vi "Modbus_RTU_Battery.vi"(0 "STOP":bool, 1 "High Volt alarm (0.01V)":string, 2 "error in":errorcluster, 3 "Low Volt alarm (0.01V)":string, 4 "Modbus RTU Address":string, 5 "Currrent Range":string(combo), 6 "VISA resource name":refnum<visa-resource-name>, 7 "baud rate":u32=9600) -> (11 "HighAlarm":bool, 13 "LowAlarm":bool, 14 "Voltage(V)":dbl, 15 "Current(A)":dbl, 16 "error out":errorcluster, 17 "Energy(Wh)":dbl, 18 "Power(W)":dbl, 19 "ChangeDone":bool)   [LabVIEW 2025]
uses:
  <vilib>/NI/Modbus Library/API/Wrapper/Create Serial Master.vi
  <vilib>/NI/Modbus Library/API/Master/Modbus Master.lvclass
  <vilib>/NI/Modbus Library/API/Wrapper/API Main.lvlib
panel:
  out "register parameter":u16[](array[numeric])
  out "register data":u16[](array[numeric])
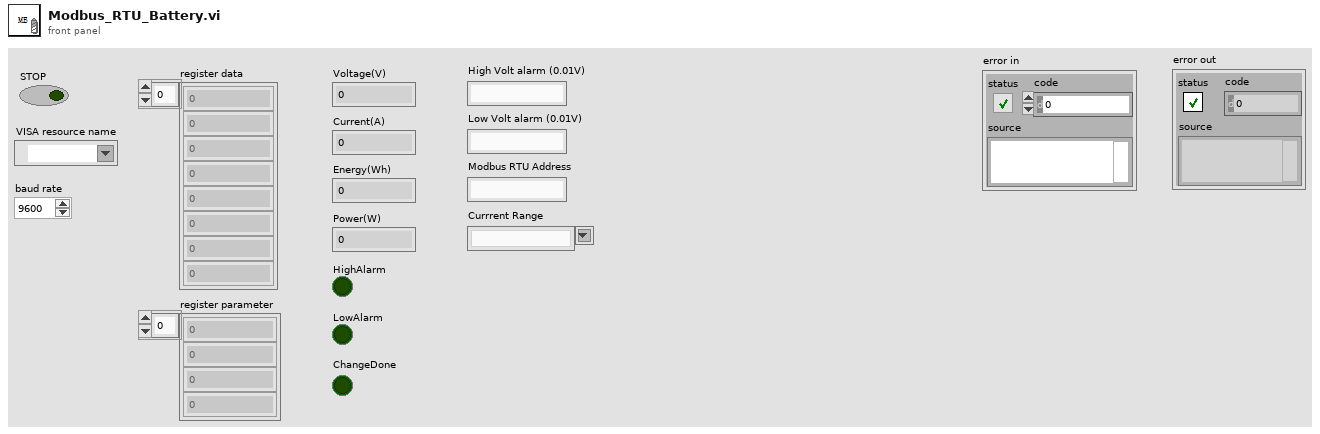
[diagram p1: front panel]
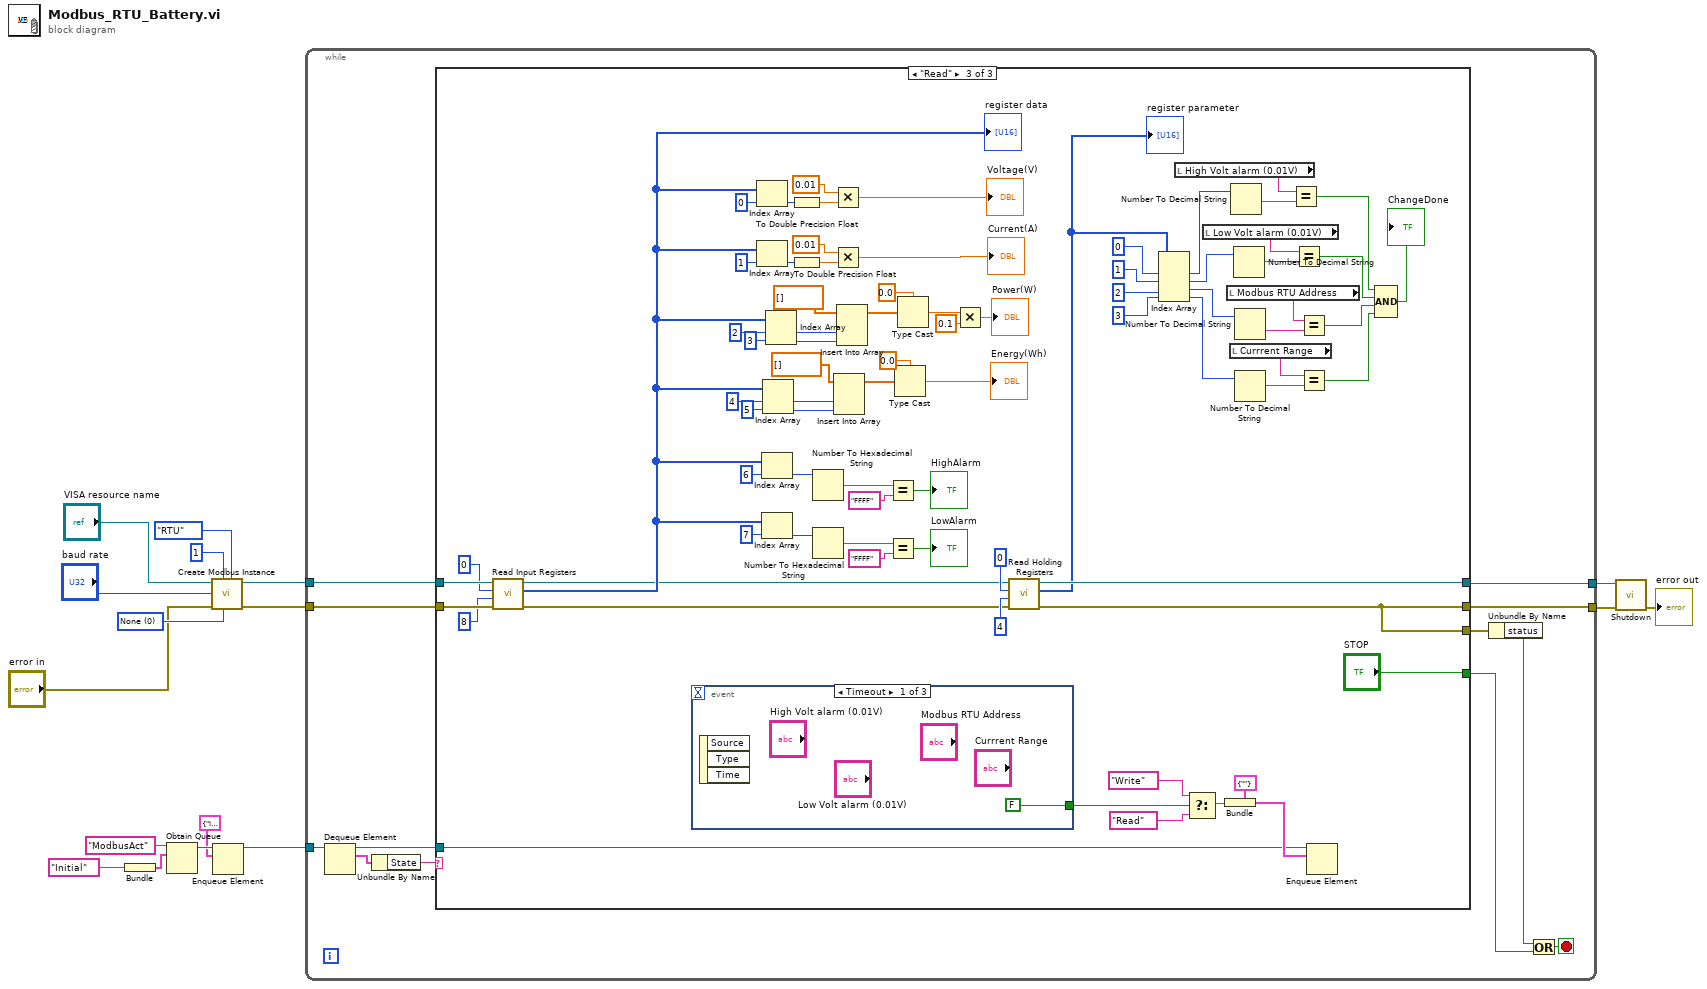
[diagram p0: block diagram]
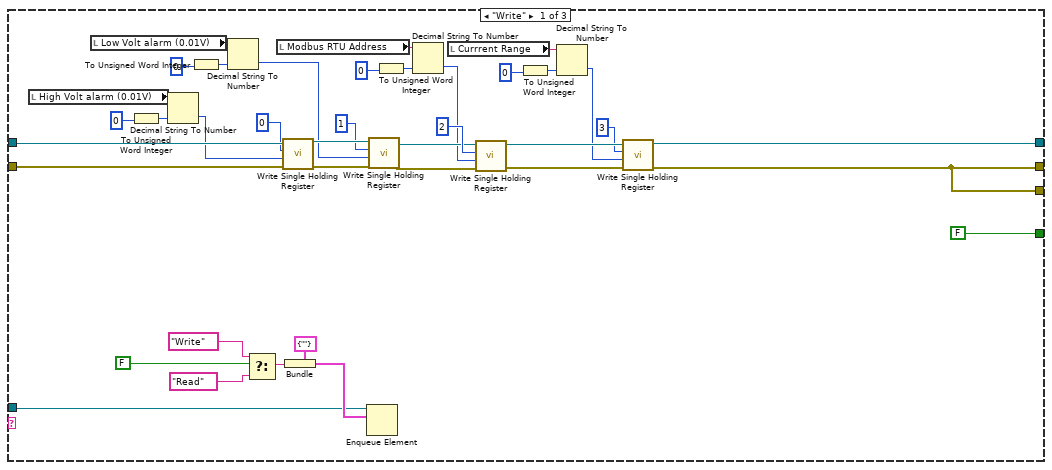
[diagram p2: hidden frame]
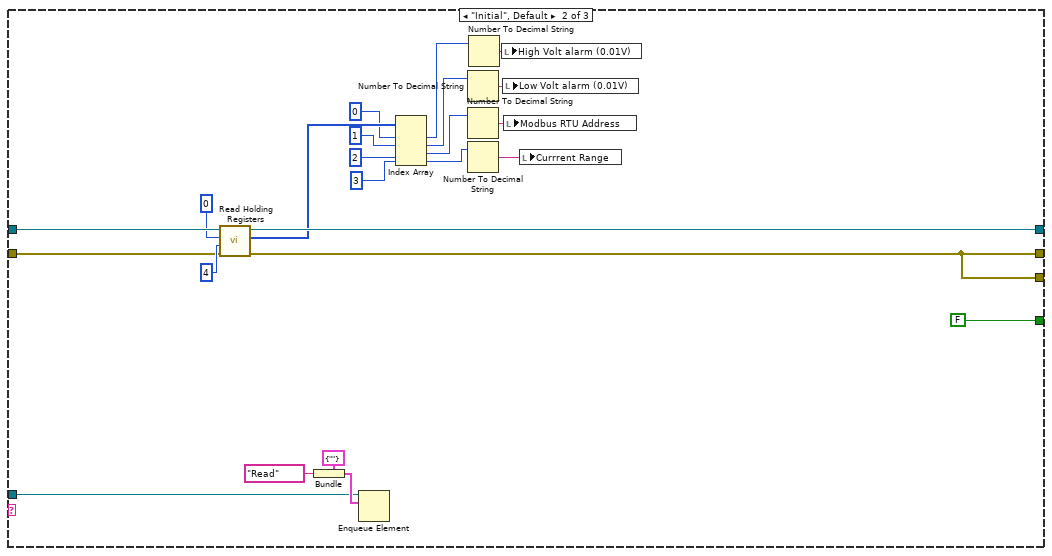
[diagram p3: hidden frame]
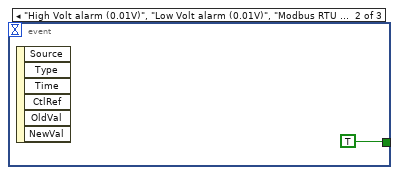
[diagram p4: hidden frame]
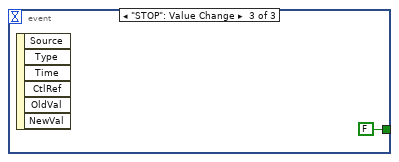
[diagram p5: hidden frame]
diagram:
  w15 = u16 0 items=["None", "Odd", "Even", "Mark", "Space"] ("parity (even)")
  n1 = Bundle("State"="Initial") -> (w6:cluster{"State":string})  [unwired: 1 in]
  n2 = Obtain Queue(name (unnamed)="ModbusAct" ("名称（未命名）"), element data type=w6) -> (queue out=w10:refnum<queue>)  [unwired: 3 in, 2 out]
  n3 = call-poly <vilib>:"Create Modbus Instance.vi"("serial type"=enum16{"RTU", "ASCII"}."RTU", "parity (even)"=w15, "unit ID"=u8 1, "error in"="error in", "baud rate"="baud rate", "VISA resource name"="VISA resource name") -> ("error out"=w13:errorcluster, "serial master instance"=w14:refnum<class "Modbus Master.lvclass">)  [unwired: 4 in]
  n4 = Enqueue Element(queue=w10, element=cluster{string} {"Initial"}) -> (queue out=w5:refnum<queue>)  [unwired: 2 in, 2 out]
  n5 = while {
    tunnel: w14 -> [w29]
    tunnel: [w27] -> w12
    tunnel: w13 -> [w28]
    tunnel: [w24] -> w11
    tunnel: w5 -> [w21]
    stop <- w26 stop-if-true
    n6 = Dequeue Element(queue=w21) -> (queue out=w20:refnum<queue>, element=w23:cluster{"State":string})  [unwired: 2 in, 2 out]
    n7 = Unbundle By Name(w23) -> ("State"=w22:string)
    n8 = case shown="\"Read\"" w22 {
      tunnel: w29 -> [w57 w85 w170]
      tunnel: w28 -> [w56 w83 w169]
      tunnel: [w32 w81 w115] -> w27
      tunnel: [w31 w82 w114] -> w24
      tunnel: w20 -> [w62 w89 w125]
      tunnel: [w31 w82 w114] -> w19
      tunnel: [FALSE ("STOP") FALSE ("STOP") "STOP"] -> w18
      frame "Write" {
        n9 = local read "High Volt alarm (0.01V)"() -> (w51:string)
        n10 = local read "Low Volt alarm (0.01V)"() -> (w50:string)
        n11 = To Unsigned Word Integer(number=0) -> (unsigned 16bit integer=w53:u16)
        n12 = Decimal String To Number(string=w51, default (0L)=w53) -> (number=w52:u16)  [unwired: 1 in, 1 out]
        n13 = To Unsigned Word Integer(number=0) -> (unsigned 16bit integer=w49:u16)
        n14 = Decimal String To Number(string=w50, default (0L)=w49) -> (number=w47:u16)  [unwired: 1 in, 1 out]
        n15 = Select(t="Write" ("State"), s=FALSE, f="Read" ("State")) -> (s? t:f=w65:string)
        n16 = local read "Modbus RTU Address"() -> (w43:string)
        n17 = call-dynamic "Write Single Holding Register.vi"("error in"=w56, "register to write"=w52, "address"=u16 0, "Modbus master in"=w57) -> ("error out"=w59:errorcluster, "Modbus master out"=w60:refnum<class "Modbus Master.lvclass">)  [unwired: 6 in]
        n18 = Bundle(cluster=cluster{string} {""}, w65) -> (w67:cluster{string})
        n19 = Enqueue Element(queue=w62, element=w67) -> ()  [unwired: 2 in, 3 out]
        n20 = call-dynamic "Write Single Holding Register.vi"("error in"=w59, "register to write"=w47, "address"=u16 1, "Modbus master in"=w60) -> ("error out"=w45:errorcluster, "Modbus master out"=w44:refnum<class "Modbus Master.lvclass">)  [unwired: 6 in]
        n21 = To Unsigned Word Integer(number=0) -> (unsigned 16bit integer=w41:u16)
        n22 = Decimal String To Number(string=w43, default (0L)=w41) -> (number=w40:u16)  [unwired: 1 in, 1 out]
        n23 = local read "Currrent Range"() -> (w35:string)
        n24 = call-dynamic "Write Single Holding Register.vi"("error in"=w45, "register to write"=w40, "address"=u16 2, "Modbus master in"=w44) -> ("error out"=w39:errorcluster, "Modbus master out"=w38:refnum<class "Modbus Master.lvclass">)  [unwired: 6 in]
        n25 = To Unsigned Word Integer(number=0) -> (unsigned 16bit integer=w37:u16)
        n26 = Decimal String To Number(string=w35, default (0L)=w37) -> (number=w33:u16)  [unwired: 1 in, 1 out]
        n27 = call-dynamic "Write Single Holding Register.vi"("error in"=w39, "register to write"=w33, "address"=u16 3, "Modbus master in"=w38) -> ("error out"=w31:errorcluster, "Modbus master out"=w32:refnum<class "Modbus Master.lvclass">)  [unwired: 6 in]
      }
      frame "Initial", Default {
        n28 = call-dynamic "Read Holding Registers.vi"("error in"=w83, "number of inputs"=u16 4, "starting address"=u16 0, "Modbus master in"=w85) -> ("error out"=w82:errorcluster, "register values"=w80:u16[], "Modbus master out"=w81:refnum<class "Modbus Master.lvclass">)  [unwired: 5 in]
        n29 = Bundle(cluster=cluster{string} {""}, "Read" ("State")) -> (w91:cluster{string})
        n30 = Enqueue Element(queue=w89, element=w91) -> ()  [unwired: 2 in, 3 out]
        n31 = Index Array(array=w80, index #1=0 ("index"), index #2=1 ("index"), index #3=2 ("index"), index #4=3 ("index")) -> (element #1=w75:u16, element #2=w72:u16, element #3=w70:u16, element #4=w68:u16)
        n32 = Number To Decimal String(number=w72) -> (decimal integer string=w73:string)  [unwired: 1 in]
        n33 = Number To Decimal String(number=w70) -> (decimal integer string=w71:string)  [unwired: 1 in]
        n34 = Number To Decimal String(number=w68) -> (decimal integer string=w69:string)  [unwired: 1 in]
        n35 = Number To Decimal String(number=w75) -> (decimal integer string=w74:string)  [unwired: 1 in]
        n36 = local write "High Volt alarm (0.01V)"(w74) -> ()
        n37 = local write "Low Volt alarm (0.01V)"(w73) -> ()
        n38 = local write "Modbus RTU Address"(w71) -> ()
        n39 = local write "Currrent Range"(w69) -> ()
      }
      frame "Read" {
        n40 = call-dynamic "Read Input Registers.vi"("error in"=w169, "number of inputs"=u16 8, "starting address"=u16 0, "Modbus master in"=w170) -> ("error out"=w116:errorcluster, "register values"=w136:u16[], "Modbus master out"=w117:refnum<class "Modbus Master.lvclass">)  [unwired: 5 in]
        "register data" <- w136
        n41 = event shown="[0] Timeout" {
          selector: _ -> [_ _ _]
          dyn-events: _ -> [_ _ _]
          timeout: _ -> [_ _ _]
          tunnel: [FALSE TRUE FALSE] -> w121
          event Timeout {
            n42 = event-data() -> ()  [unwired: 1 in, 3 out]
          }
          event "High Volt alarm (0.01V)", "Low Volt alarm (0.01V)", "Modbus RTU Address", "Currrent Range": Value Change {
            n43 = event-data() -> ()  [unwired: 1 in, 6 out]
          }
          event "STOP": Value Change {
            n44 = event-data() -> ()  [unwired: 1 in, 6 out]
          }
        }
        n45 = Index Array(array=w136, index=0) -> (element=w147:u16)
        n46 = Index Array(array=w136, index=1) -> (element=w141:u16)
        n47 = Index Array(array=w136, index=6) -> (element=w128:u16)
        n48 = Index Array(array=w136, index=7) -> (element=w135:u16)
        n49 = Index Array(array=w136, index #1=4 ("index"), index #2=5 ("index")) -> (element #1=w163:u16, element #2=w164:u16)
        n50 = Index Array(array=w136, index #1=2 ("index"), index #2=3 ("index")) -> (element #1=w154:u16, element #2=w153:u16)
        n51 = To Double Precision Float(number=w147) -> (double precision float=w146:dbl)
        n52 = To Double Precision Float(number=w141) -> (double precision float=w142:dbl)
        n53 = Number To Hexadecimal String(2:w128) -> (0:w129:string)  [unwired: 1 in]
        n54 = Number To Hexadecimal String(2:w135) -> (0:w134:string)  [unwired: 1 in]
        n55 = Multiply(x=0.01, y=w146) -> (x*y=→"Voltage(V)":dbl)
        n56 = Multiply(x=0.01, y=w142) -> (x*y=→"Current(A)":dbl)
        n57 = Insert Into Array(array=dbl[] [], new element #1=w163, new element #2=w164) -> (w165:dbl[])  [unwired: 1 in]
        n58 = Insert Into Array(array=dbl[] [], new element #1=w154, new element #2=w153) -> (w152:dbl[])  [unwired: 1 in]
        n59 = Equal?(x=w129, y="FFFF") -> (x = y?=→"HighAlarm":bool)
        n60 = Equal?(x=w134, y="FFFF") -> (x = y?=→"LowAlarm":bool)
        n61 = Type Cast(type=0.0, x=w165) -> (*(type *) &x=→"Energy(Wh)":dbl)
        n62 = Type Cast(type=0.0, x=w152) -> (*(type *) &x=w150:dbl)
        n63 = Multiply(x=w150, y=0.1) -> (x*y=→"Power(W)":dbl)
        n64 = call-dynamic "Read Holding Registers.vi"("error in"=w116, "number of inputs"=u16 4, "starting address"=u16 0, "Modbus master in"=w117) -> ("error out"=w114:errorcluster, "register values"=w105:u16[], "Modbus master out"=w115:refnum<class "Modbus Master.lvclass">)  [unwired: 5 in]
        "register parameter" <- w105
        n65 = Index Array(array=w105, index #1=0 ("index"), index #2=1 ("index"), index #3=2 ("index"), index #4=3 ("index")) -> (element #1=w109:u16, element #2=w108:u16, element #3=w107:u16, element #4=w106:u16)
        n66 = local read "High Volt alarm (0.01V)"() -> (w103:string)
        n67 = Select(t="Write" ("State"), s=w121, f="Read" ("State")) -> (s? t:f=w124:string)
        n68 = local read "Low Volt alarm (0.01V)"() -> (w101:string)
        n69 = Bundle(cluster=cluster{string} {""}, w124) -> (w127:cluster{string})
        n70 = local read "Modbus RTU Address"() -> (w100:string)
        n71 = local read "Currrent Range"() -> (w97:string)
        n72 = Number To Decimal String(number=w109) -> (decimal integer string=w104:string)  [unwired: 1 in]
        n73 = Number To Decimal String(number=w108) -> (decimal integer string=w102:string)  [unwired: 1 in]
        n74 = Number To Decimal String(number=w107) -> (decimal integer string=w99:string)  [unwired: 1 in]
        n75 = Number To Decimal String(number=w106) -> (decimal integer string=w98:string)  [unwired: 1 in]
        n76 = Equal?(x=w103, y=w104) -> (x = y?=w96:bool)
        n77 = Equal?(x=w101, y=w102) -> (x = y?=w95:bool)
        n78 = Equal?(x=w100, y=w99) -> (x = y?=w94:bool)
        n79 = Equal?(x=w97, y=w98) -> (x = y?=w93:bool)
        n80 = Enqueue Element(queue=w125, element=w127) -> ()  [unwired: 2 in, 3 out]
        n81 = Compound Arithmetic op=AND(w96, w95, w94, w93) -> (→"ChangeDone":bool)
      }
    }
    n82 = Unbundle By Name(w19) -> ("status"=w25:bool)
    n83 = Or(x=w25, y=w18) -> (x .or. y?=w26:bool)
  }
  n84 = call-dynamic "Shutdown.vi"("error in"=w11, "Modbus master in"=w12) -> ("error out"=→"error out":errorcluster)  [unwired: 9 in]
